vi "Is An Event Frame.vi"(7 "Event Structure index":i32, 10 "index of element":i32, 11 "Num Event Frames":i32) -> (2 "Structure Type":T1, 3 "Event Frame?":bool)   [LabVIEW 2020]
uses:
  StructureTypes.ctl
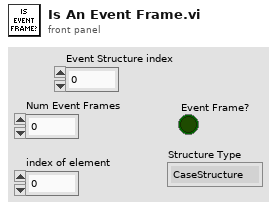
[diagram p1: front panel]
types:
  T1 = typedef "StructureTypes.ctl" = enum16{"CaseStructure", "EventStructure"}
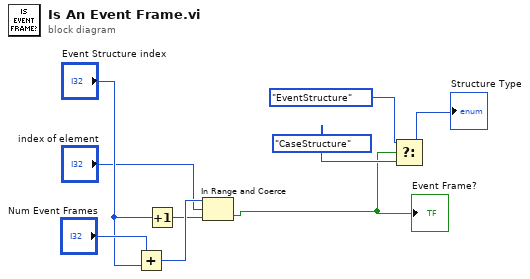
[diagram p0: block diagram]
diagram:
  n1 = Add(x="Num Event Frames", y="Event Structure index") -> (x+y=w4:i32)
  n2 = Increment(x="Event Structure index") -> (x+1=w1:i32)
  n3 = In Range and Coerce(upper limit=w4, x="index of element", lower limit=w1) -> (In Range?=w2:bool)  [unwired: 1 out]
  "Event Frame?" <- w2
  n4 = Select(t=StructureTypes."EventStructure" ("Structure Type"), s=w2, f=StructureTypes."CaseStructure" ("Structure Type")) -> (s? t:f=→"Structure Type":T1)
